vi "FuncVI_Sub - Probe - Master.vi"() -> ()   [LabVIEW 2021]
doc: "::: CalcExpress Toolkit :::\nCopyright (c) 2000-2026 Konstantin Shifershteyn. All rights reserved."
uses:
  cetypes.llb/CalcExpress Function Argument Info.ctl
  <vilib>/Utility/miscctls.llb/LVPointTypeDef.ctl
panel:
  out "I32B":i32 caption="Bit-keeping conversion" format="%.0x"
  in  "EnaWrap":bool=TRUE caption="Wrap Text"
  in  "ShowInt32":bool caption="show I32"
  out "I32M":i32 caption="Saturating conversion" format="%.0x"
  out "Index Range":cluster{"Initial index":i32, "Final index":i32}
  out "flattened data":string
  out "a2str":string[][](array[string])
  out "a1str":string[](array[string])
  out "a2cdb":cdb[][](array[numeric]) format="%.2f"
  out "a1cdb":cdb[](array[numeric]) format="%.2f"
  out "dbl":dbl format="%.2f"
  in  "update":bool
  in  "arg":T1
  out "a2dbl":dbl[][](array[numeric]) format="%.2f"
  out "cdb":cdb format="%.2f"
  out "a1dbl":dbl[](array[numeric]) format="%.2f"
  in  "Display style":u32(ring) items=["Normal", "'\\' Code", "Password", "Hex dump"]
  out "str":string
  in  "Precision":u8=3
  in  "Format":u8(ring) items=["Floating point", "Scientific", "Engineering", "Binary", "Octal", "Hexadecimal", "Relative time", "Absolute time"]
  out "datatype":u32(ring)=10 items=["String"=0, "DBL Number"=1, "Identifier"=2, "1D Array of DBL"=3, "2D Array of DBL"=4, "CDB Number"=5, "1D Array of CDB"=6, "2D Array of CDB"=7, "1D Array of String"=8, "2D Array of String"=9, "Unknown data type"=10, "Index Range"=252]
  # "Value:"
  # ":"
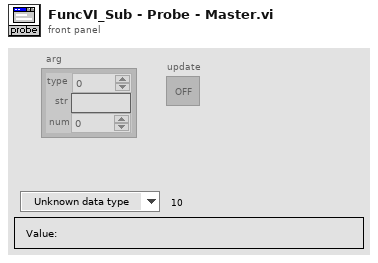
[diagram p1: front panel]
types:
  T1 = typedef "CalcExpress Function Argument Info.ctl" = cluster{"type":u32, "str":string, "num":dbl}
  T2 = typedef "LVPointTypeDef.ctl" = cluster{"Horizontal":i16, "Vertical":i16}
  T3 = typedef "eventvkey.ctl" = enum16{"ASCII", "Enter", "Return", "Shift", "Ctrl", "Alt", "Cmd", "Opt", "Caps", "NumLock", "Clear", "Break", "Up", "Down", "Left", "Right", "Insert", "Delete", "Home", "End", "PageUp", "PageDown", "Escape", "Help", "Pause", "ScrollLock", "F1", "F2", "F3", "F4", "F5", "F6", "F7", "F8", "F9", "F10", "F11", "F12", "F13", "F14", "F15", "F16", "F17", "F18", "F19", "F20", "F21", "F22", "F23", "F24", "Play", "VolumeUp", "VolumeDown", "Mute", "Two Byte Char"}
  T4 = cluster{"Shift":bool, "Ctrl":bool, "Alt":bool, "Cmd":bool, "Opt":bool}
  T5 = typedef "LVRectTypeDef.ctl" = cluster{"Left":i16, "Top":i16, "Right":i16, "Bottom":i16}
  T6 = cluster{"Left":i32, "Top":i32, "Right":i32, "Bottom":i32}
  T7 = typedef "LVPositionTypeDef.ctl" = cluster{"Left":i32, "Top":i32}
  T8 = typedef "LVBoundsTypeDef.ctl" = cluster{"Width":u32, "Height":u32}
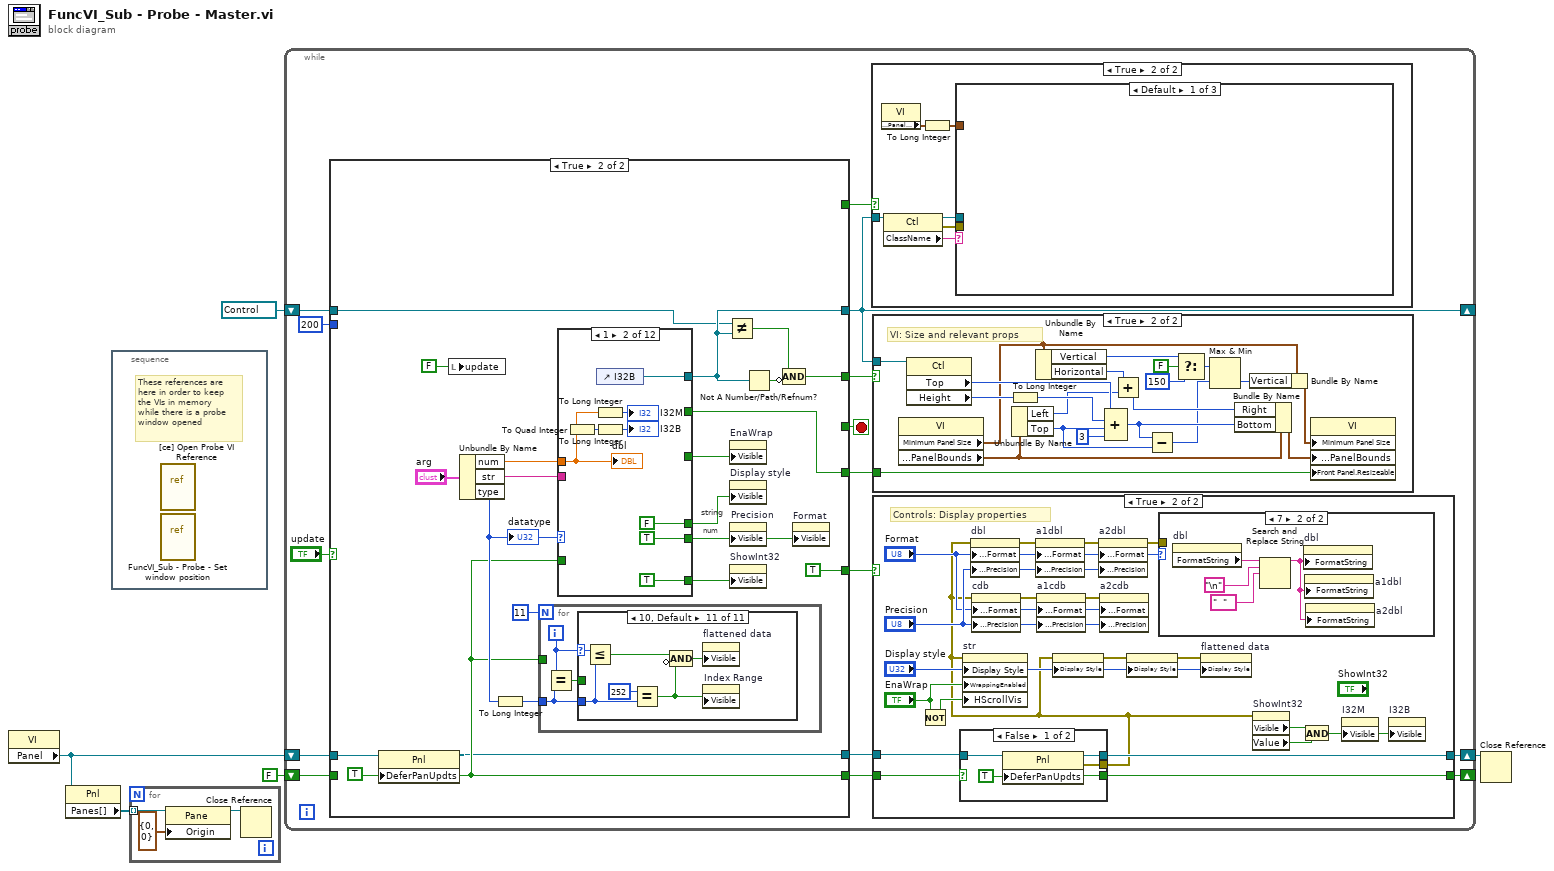
[diagram p0: block diagram]
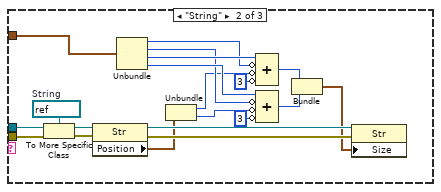
[diagram p3: hidden frame]
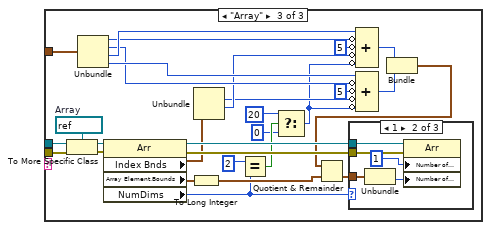
[diagram p4: hidden frame]
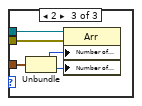
[diagram p6: hidden frame]
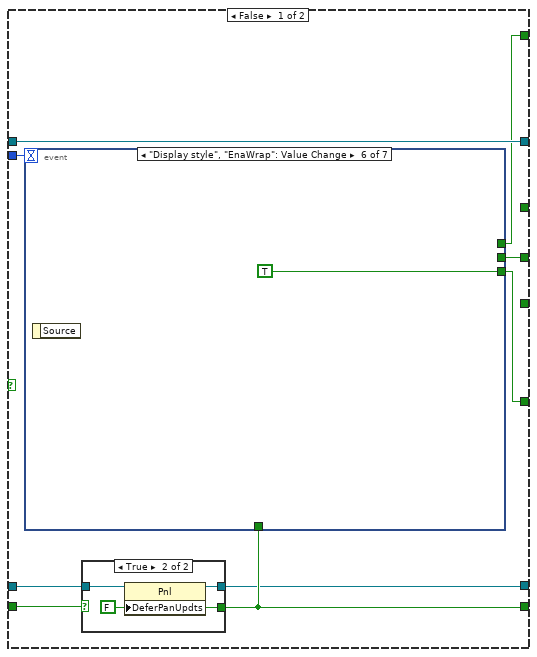
[diagram p8: hidden frame]
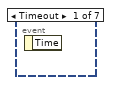
[diagram p10: hidden frame]
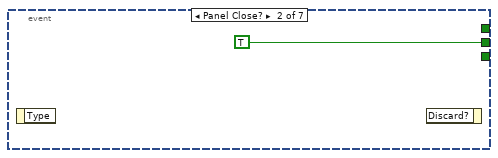
[diagram p11: hidden frame]
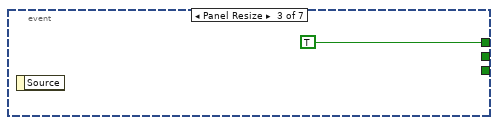
[diagram p12: hidden frame]
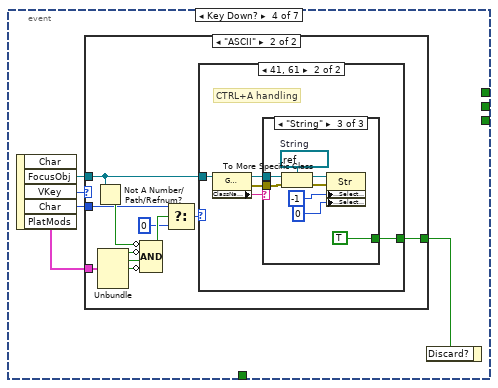
[diagram p13: hidden frame]
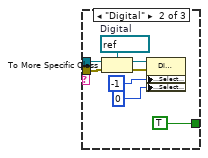
[diagram p17: hidden frame]
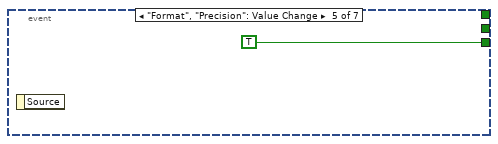
[diagram p18: hidden frame]
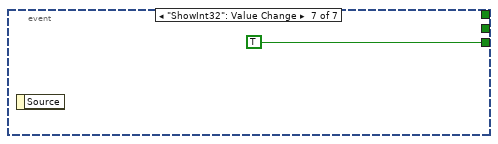
[diagram p19: hidden frame]
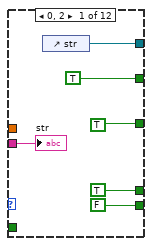
[diagram p20: hidden frame]
diagram:
  n1 = property on="Property Node" class="VI"() -> ("Panel"=w4:refnum<vi>)  [unwired: 2 in, 2 out]
  n2 = property on="Property Node" class="Pnl"(reference=w4) -> ("Panes[]"=w2:refnum<vi>[])  [unwired: 1 in, 2 out]
  n3 = stacked-sequence {
    frame #0 {
      # "These references are\nhere in order to keep\nthe VIs in memory\nwhile there is a probe\nwindow opened"
      n4 = vi-ref "[ce] Open Probe VI Reference.vi"() -> ()  [unwired: 1 out]
      n5 = vi-ref "FuncVI_Sub - Probe - Set window position.vi"() -> ()  [unwired: 1 out]
    }
  }
  n6 = for {
    tunnel: w2 -> [w8] mode=indexing
    n7 = property on="Property Node" class="Pane"(reference=w8, "Origin"=T2 {"Horizontal"=0, "Vertical"=0}) -> (reference out=w6:refnum<vi>)  [unwired: 1 in, 1 out]
    n8 = Close Reference(reference=w6) -> ()  [unwired: 1 in, 1 out]
  }
  n9 = while {
    shift-right: [w16] -> _
    shift-left: refnum<vi> refnum ("int32") -> [w18]
    shift-right: [w13] -> _
    shift-left: FALSE ("Defer Panel Updates") -> [w14]
    shift-right: [w10] -> w3
    shift-left: w4 -> [w15]
    stop <- w22 stop-if-true
    n10 = case shown="True" "update" {
      tunnel: [w118 _] -> w22
      tunnel: [w117 TRUE] -> w21
      tunnel: [w116 w173] -> w16
      tunnel: [_ w176] -> w20
      tunnel: [_ w174] -> w19
      tunnel: w18 -> [w116 w172]
      tunnel: [w115 _] -> w17
      tunnel: [w112 w169] -> w12
      tunnel: w15 -> [w114 w170]
      tunnel: w14 -> [w113 _]
      tunnel: [w111 w168] -> w11
      tunnel: 200 -> [w110 _]
      frame False {
        n11 = case shown="True" w113 {
          selector: w113 -> [w120 _]
          tunnel: w114 -> [w119 w123]
          tunnel: [w120 w122] -> w112
          tunnel: [w119 w121] -> w111
          frame False {
          }
          frame True {
            w122 = FALSE ("Defer Panel Updates")
            n12 = property on="Property Node" class="Pnl"(reference=w123, "DeferPanUpdts"=w122) -> (reference out=w121:refnum<vi>)  [unwired: 1 in, 1 out]
          }
        }
        n13 = event shown="[5] \"Display style\", \"EnaWrap\": Value Change" {
          selector: _ -> [_ _ _ _ _ _ _]
          dyn-events: _ -> [_ _ _ _ _ _ _]
          timeout: w110 -> [_ _ _ _ _ _ _]
          tunnel: [_ TRUE _ _ _ _ _] -> w118
          tunnel: [_ _ _ _ TRUE TRUE TRUE] -> w117
          tunnel: [_ _ TRUE _ _ _ _] -> w115
          tunnel: w112 -> [_ _ _ _ _ _ _]
          event Timeout {
            n14 = event-data() -> ()  [unwired: 1 in, 1 out]
          }
          event Panel Close? {
            n15 = event-data() -> ()  [unwired: 1 in, 1 out]
            n16 = event-data ("Event Filter Node")() -> ()  [unwired: 2 in, 1 out]
          }
          event Panel Resize {
            n17 = event-data() -> ()  [unwired: 1 in, 1 out]
          }
          event Key Down? {
            n18 = event-data() -> ("FocusObj"=w128:refnum<vi>, "VKey"=w130:T3, "Char"=w127:i16, "PlatMods"=w129:T4)  [unwired: 1 in, 1 out]
            n19 = case shown="\"ASCII\"" w130 {
              tunnel: w129 -> [_ w137]
              tunnel: w128 -> [_ w136]
              tunnel: w127 -> [_ w135]
              tunnel: [_ w131] -> w126
              frame Default {
              }
              frame "ASCII" {
                n20 = Not A Number/Path/Refnum?(number/path/refnum=w136) -> (NaN/Path/Refnum?=w138:bool)
                n21 = Unbundle(w137) -> ("Shift"=w139:bool, "Ctrl"=w140:bool, "Alt"=w141:bool)  [unwired: 2 out]
                n22 = Compound Arithmetic op=AND(invert w138, invert w139, w140, invert w141) -> (w134:bool)
                n23 = Select(t=w135, s=w134, f=i16 0) -> (s? t:f=w132:i16)
                n24 = case shown="41, 61" w132 {
                  tunnel: w136 -> [_ w146]
                  tunnel: [_ w142] -> w131
                  frame Default {
                  }
                  frame 65, 97 {
                    # "CTRL+A handling"
                    n25 = property on="Property Node" class="GObj"(reference=w146) -> (reference out=w144:refnum<vi>, error out=w143:errorcluster, "ClassName"=w145:string)  [unwired: 1 in]
                    n26 = case shown="\"String\"" w145 {
                      tunnel: w144 -> [_ w150 w158]
                      tunnel: w143 -> [_ w149 w157]
                      tunnel: [_ TRUE TRUE] -> w142
                      frame Default {
                      }
                      frame "Digital" {
                        w151 = refnum<vi> refnum  # Digital
                        n27 = To More Specific Class(target class=w151, reference=w150, error in=w149) -> (specific class reference=w154:refnum<vi>, error out=w148:errorcluster)
                        n28 = property on="Property Node" class="DigNum"(reference=w154, error in=w148, "NumText.Selection End"=-1 ("Numeric Text.Selection:End"), "NumText.Selection Start"=u32 0 ("Numeric Text.Selection:Start")) -> ()  [unwired: 2 out]
                      }
                      frame "String" {
                        w159 = refnum<vi> refnum  # String
                        n29 = To More Specific Class(target class=w159, reference=w158, error in=w157) -> (specific class reference=w162:refnum<vi>, error out=w156:errorcluster)
                        n30 = property on="Property Node" class="Str"(reference=w162, error in=w156, "Text.Selection End"=-1 ("Numeric Text.Selection:End"), "Text.Selection Start"=u32 0 ("Numeric Text.Selection:Start")) -> ()  [unwired: 2 out]
                      }
                    }
                  }
                }
              }
            }
            n31 = event-data ("Event Filter Node")("Discard?"=w126) -> ()  [unwired: 1 in, 1 out]
          }
          event "Format", "Precision": Value Change {
            n32 = event-data() -> ()  [unwired: 1 in, 1 out]
          }
          event "Display style", "EnaWrap": Value Change {
            n33 = event-data() -> ()  [unwired: 1 in, 1 out]
          }
          event "ShowInt32": Value Change {
            n34 = event-data() -> ()  [unwired: 1 in, 1 out]
          }
        }
      }
      frame True {
        w169 = TRUE
        # "num"
        # "string"
        n35 = property on="Property Node" class="Pnl"(reference=w170, "DeferPanUpdts"=w169) -> (reference out=w168:refnum<vi>)  [unwired: 1 in, 1 out]
        n36 = local write "update"(FALSE ("update")) -> ()
        n37 = Unbundle By Name("arg") -> ("num"=w184:dbl, "str"=w185:string, "type"=w179:u32)
        "datatype" <- w179
        n38 = To Long Integer(number=w179) -> (32bit integer=w183:i32)
        n39 = for {
          N: 11 -> [_]
          tunnel: w183 -> [w262]
          tunnel: w169 -> [_]
          i -> [w263]
          n40 = Equal?(x=w263, y=w262) -> (x = y?=w264:bool)
          n41 = case shown="10, Default" w263 {
            selector: w263 -> [_ _ _ _ _ _ _ _ _ _ w279]
            tunnel: w264 -> [w265 w266 _ w267 w268 w269 w270 w271 w272 w273 _]
            tunnel: w262 -> [_ _ _ _ _ _ _ _ _ _ w278]
            frame 0 {
              n42 = property on="str" class="Str"("Visible"=w265) -> ()  [unwired: 2 in, 2 out]
            }
            frame 1 {
              n43 = property on="dbl" class="DigNum (strict)"("Visible"=w266) -> ()  [unwired: 2 in, 2 out]
            }
            frame 2 {
            }
            frame 3 {
              n44 = property on="a1dbl" class="Arr (strict)"("Visible"=w267) -> ()  [unwired: 2 in, 2 out]
            }
            frame 4 {
              n45 = property on="a2dbl" class="Arr (strict)"("Visible"=w268) -> ()  [unwired: 2 in, 2 out]
            }
            frame 5 {
              n46 = property on="cdb" class="DigNum (strict)"("Visible"=w269) -> ()  [unwired: 2 in, 2 out]
            }
            frame 6 {
              n47 = property on="a1cdb" class="Arr (strict)"("Visible"=w270) -> ()  [unwired: 2 in, 2 out]
            }
            frame 7 {
              n48 = property on="a2cdb" class="Arr (strict)"("Visible"=w271) -> ()  [unwired: 2 in, 2 out]
            }
            frame 8 {
              n49 = property on="a1str" class="Arr (strict)"("Visible"=w272) -> ()  [unwired: 2 in, 2 out]
            }
            frame 9 {
              n50 = property on="a2str" class="Arr (strict)"("Visible"=w273) -> ()  [unwired: 2 in, 2 out]
            }
            frame 10, Default {
              n51 = Less Or Equal?(x=w279, y=w278) -> (x <= y?=w274:bool)
              n52 = Equal?(x=252, y=w278) -> (x = y?=w275:bool)
              n53 = Compound Arithmetic op=AND(w274, invert w275) -> (w276:bool)
              n54 = property on="flattened data" class="Str"("Visible"=w276) -> ()  [unwired: 2 in, 2 out]
              n55 = property on="Index Range" class="Clust (strict)"("Visible"=w275) -> ()  [unwired: 2 in, 2 out]
            }
          }
        }
        n56 = case shown="1" w179 {
          tunnel: w184 -> [_ w193 _ _ _ _ _ _ _ _ _ w261]
          tunnel: [FALSE TRUE FALSE TRUE TRUE TRUE TRUE TRUE FALSE FALSE FALSE FALSE] -> w181
          tunnel: [TRUE FALSE FALSE FALSE FALSE FALSE FALSE FALSE TRUE TRUE TRUE FALSE] -> w167
          tunnel: w185 -> [w190 _ _ w208 w215 w221 w228 w234 w242 w248 w254 _]
          tunnel: [_ TRUE _ _ _ _ _ _ _ _ _ _] -> w177
          tunnel: [w189 w196 refnum<vi> refnum ("int32") w205 w212 w218 w225 w232 w239 w246 w253 w257] -> w173
          tunnel: [TRUE _ _ TRUE TRUE _ TRUE TRUE TRUE TRUE TRUE _] -> w174
          tunnel: w169 -> [_ _ _ _ _ _ _ _ _ _ _ _]
          tunnel: [TRUE _ _ _ _ _ _ _ _ _ _ _] -> w166
          frame 0, 2 {
            n57 = control-ref of="str"() -> (w189:refnum<vi>)
            "str" <- w190
          }
          frame 1 {
            n58 = To Quad Integer(1:w193) -> (0:w194:i64)
            n59 = To Long Integer(number=w193) -> (32bit integer=→"I32M":i32)
            n60 = To Long Integer(number=w194) -> (32bit integer=→"I32B":i32)
            n61 = control-ref of="I32B"() -> (w196:refnum<vi>)
            "dbl" <- w193
          }
          frame 22222 {
          }
          frame 3 {
            n62 = control-ref of="a1dbl"() -> (w205:refnum<vi>)
            n63 = Unflatten From String(type=dbl[] [] ("a1dbl"), binary string=w208) -> (value=→"a1dbl":dbl[])  [unwired: 3 in, 2 out]
          }
          frame 4 {
            n64 = control-ref of="a2dbl"() -> (w212:refnum<vi>)
            n65 = Unflatten From String(type=dbl[][] [] ("a1dbl"), binary string=w215) -> (value=→"a2dbl":dbl[][])  [unwired: 3 in, 2 out]
          }
          frame 5 {
            n66 = control-ref of="cdb"() -> (w218:refnum<vi>)
            n67 = Unflatten From String(type=cdb 0.0+0.0i ("cdb"), binary string=w221) -> (value=→"cdb":cdb)  [unwired: 3 in, 2 out]
          }
          frame 6 {
            n68 = control-ref of="a1cdb"() -> (w225:refnum<vi>)
            n69 = Unflatten From String(type=cdb[] [] ("a1dbl"), binary string=w228) -> (value=→"a1cdb":cdb[])  [unwired: 3 in, 2 out]
          }
          frame 7 {
            n70 = Unflatten From String(type=cdb[][] [] ("a1dbl"), binary string=w234) -> (value=→"a2cdb":cdb[][])  [unwired: 3 in, 2 out]
            n71 = control-ref of="a2cdb"() -> (w232:refnum<vi>)
          }
          frame 8 {
            n72 = control-ref of="a1str"() -> (w239:refnum<vi>)
            n73 = Unflatten From String(type=string[] [] ("a1str"), binary string=w242) -> (value=→"a1str":string[])  [unwired: 3 in, 2 out]
          }
          frame 9 {
            n74 = control-ref of="a2str"() -> (w246:refnum<vi>)
            n75 = Unflatten From String(type=string[][] [] ("a1str"), binary string=w248) -> (value=→"a2str":string[][])  [unwired: 3 in, 2 out]
          }
          frame 10, Default {
            n76 = control-ref of="flattened data"() -> (w253:refnum<vi>)
            "flattened data" <- w254
          }
          frame 252 {
            n77 = call "[ce] Index Range to-from DBL.vi"("dbl scalar"=w261) -> ("Index Range out"=→"Index Range":cluster{"Initial index":i32, "Final index":i32})  [unwired: 9 in, 1 out]
            n78 = control-ref of="Index Range"() -> (w257:refnum<vi>)
          }
        }
        n79 = Not Equal?(x=w172, y=w173) -> (x != y?=w171:bool)
        n80 = property on="EnaWrap" class="Bool (strict)"("Visible"=w166) -> ()  [unwired: 2 in, 2 out]
        n81 = property on="Display style" class="Ring (strict)"("Visible"=w167) -> ()  [unwired: 2 in, 2 out]
        n82 = property on="Precision" class="DigNum (strict)"("Visible"=w181) -> ()  [unwired: 2 in, 2 out]
        n83 = property on="ShowInt32" class="Bool (strict)"("Visible"=w177) -> ()  [unwired: 2 in, 2 out]
        n84 = Not A Number/Path/Refnum?(number/path/refnum=w173) -> (NaN/Path/Refnum?=w175:bool)
        n85 = Compound Arithmetic op=AND(w171, invert w175) -> (w176:bool)
        n86 = property on="Format" class="Ring (strict)"("Visible"=w181) -> ()  [unwired: 2 in, 2 out]
      }
    }
    n87 = case shown="True" w17 {
      tunnel: w16 -> [_ w29]
      frame False {
      }
      frame True {
        n88 = property on="Property Node" class="VI"() -> ("Front Panel.PanelBounds"=w25:T5)  [unwired: 2 in, 2 out]
        n89 = property on="Property Node" class="Ctl"(reference=w29) -> (reference out=w27:refnum<vi>, error out=w26:errorcluster, "ClassName"=w28:string)  [unwired: 1 in]
        n90 = To Long Integer(number=w25) -> (32bit integer=w24:T6)
        n91 = case shown="Default" w28 {
          tunnel: w27 -> [_ w49 w78]
          tunnel: w26 -> [_ w34 w69]
          tunnel: w24 -> [_ w31 w66]
          frame Default {
          }
          frame "String" {
            w48 = refnum<vi> refnum  # String
            n92 = To More Specific Class(target class=w48, reference=w49, error in=w34) -> (specific class reference=w33:refnum<vi>, error out=w32:errorcluster)
            n93 = property on="Property Node" class="Str"(reference=w33, error in=w32) -> (reference out=w46:refnum<vi>, error out=w47:errorcluster, "Position"=w45:T7)
            n94 = Unbundle(w31) -> ("Left"=w30:i32, "Top"=w42:i32, "Right"=w44:i32, "Bottom"=w43:i32)
            n95 = Unbundle(w45) -> ("Left"=w41:i32, "Top"=w40:i32)
            n96 = Compound Arithmetic op=ADD(w44, invert w30, invert w41, invert 3 ("value")) -> (w39:i32)
            n97 = Compound Arithmetic op=ADD(w43, invert w42, invert w40, invert 3 ("value")) -> (w38:i32)
            n98 = Bundle(w39, w38) -> (w37:cluster{i32, i32})  [unwired: 1 in]
            n99 = property on="Property Node" class="Str"(reference=w46, error in=w47, "Size"=w37) -> ()  [unwired: 2 out]
          }
          frame "Array" {
            w77 = refnum<vi> refnum  # Array
            n100 = To More Specific Class(target class=w77, reference=w78, error in=w69) -> (specific class reference=w68:refnum<vi>, error out=w67:errorcluster)
            n101 = Unbundle(w66) -> ("Left"=w65:i32, "Top"=w72:i32, "Right"=w74:i32, "Bottom"=w73:i32)
            n102 = property on="Property Node" class="Arr"(reference=w68, error in=w67) -> (reference out=w75:refnum<vi>, error out=w76:errorcluster, "Index Bnds"=w59:T5, "Array Element.Bounds"=w64:T8, "NumDims"=w51:u32)
            n103 = To Long Integer(number=w64) -> (32bit integer=w61:cluster{"Width":i32, "Height":i32})
            n104 = Unbundle(w59) -> ("Top"=w57:i16, "Right"=w58:i16)  [unwired: 2 out]
            n105 = Equal?(x=u32 2 ("y"), y=w51) -> (x = y?=w55:bool)
            n106 = Select(t=20 ("value"), s=w55, f=0) -> (s? t:f=w50:i32)
            n107 = Compound Arithmetic op=ADD(w74, invert w65, invert 5 ("value"), invert w58, invert w50) -> (w71:i32)
            n108 = Compound Arithmetic op=ADD(w73, invert w72, invert 5 ("value"), invert w57, invert w50) -> (w70:i32)
            n109 = Bundle(w71, w70) -> (w56:cluster{i32, i32})  [unwired: 1 in]
            n110 = Quotient & Remainder(x=w56, y=w61) -> (floor(x/y)=w60:cluster{i32, i32})  [unwired: 1 out]
            n111 = case shown="1" w51 {
              tunnel: w76 -> [_ w83 w88]
              tunnel: w75 -> [_ w82 w87]
              tunnel: w60 -> [_ w81 w86]
              frame 0, Default {
              }
              frame 1 {
                n112 = Unbundle(w81) -> (w80:i32)  [unwired: 1 out]
                n113 = property on="Property Node" class="Arr"(reference=w82, error in=w83, "Number of Columns"=u32 1, "Number of Rows"=w80) -> ()  [unwired: 2 out]
              }
              frame 2 {
                n114 = Unbundle(w86) -> (w85:i32, w84:i32)
                n115 = property on="Property Node" class="Arr"(reference=w87, error in=w88, "Number of Columns"=w85, "Number of Rows"=w84) -> ()  [unwired: 2 out]
              }
            }
          }
        }
      }
    }
    n116 = case shown="True" w20 {
      tunnel: w16 -> [_ w109]
      tunnel: w19 -> [_ w97]
      frame False {
      }
      frame True {
        # "VI: Size and relevant props"
        n117 = property on="Property Node" class="VI"() -> ("Minimum Panel Size"=w96:T2, "Front Panel.PanelBounds"=w104:T5)  [unwired: 2 in, 2 out]
        n118 = property on="Property Node" class="Ctl"(reference=w109) -> ("Top"=w108:i32, "Height"=w107:u32)  [unwired: 1 in, 2 out]
        n119 = To Long Integer(number=w107) -> (32bit integer=w106:i32)
        n120 = Unbundle By Name(w104) -> ("Left"=w101:i16, "Top"=w98:i16)
        n121 = Unbundle By Name(w96) -> ("Vertical"=w92:i16, "Horizontal"=w102:i16)
        n122 = Compound Arithmetic op=ADD(w108, w106, w98, 3 ("value")) -> (w99:i32)
        n123 = Add(x=w102, y=w101) -> (x+y=w100:i16)
        n124 = Subtract(x=w99, y=w98) -> (x-y=w93:i32)
        n125 = Select(t=w92, s=FALSE, f=150 ("x")) -> (s? t:f=w90:i32)
        n126 = Max & Min(x=w90, y=w93) -> (min(x,y)=w94:i32)  [unwired: 1 out]
        n127 = Bundle By Name(cluster=w104, "Right"=w100, "Bottom"=w99) -> (w103:T5)
        n128 = Bundle By Name(cluster=w96, "Vertical"=w94) -> (w95:T2)
        n129 = property on="Property Node" class="VI"("Minimum Panel Size"=w95, "Front Panel.PanelBounds"=w103, "Front Panel.Resizeable"=w97) -> ()  [unwired: 2 in, 2 out]
      }
    }
    n130 = case shown="True" w21 {
      tunnel: [w281 w293] -> w13
      tunnel: w12 -> [w281 w294]
      tunnel: w11 -> [w280 w295]
      tunnel: [w280 w284] -> w10
      frame False {
      }
      frame True {
        # "Controls: Display properties"
        n131 = Not(x="EnaWrap") -> (.not. x?=w285:bool)
        n132 = case shown="False" w294 {
          selector: w294 -> [_ w307]
          tunnel: w295 -> [w305 w306]
          tunnel: [w304 w307] -> w293
          tunnel: [w303 w306] -> w284
          tunnel: [w302 _] -> w283
          frame False {
            w304 = TRUE ("Defer Panel Updates")
            n133 = property on="Property Node" class="Pnl"(reference=w305, "DeferPanUpdts"=w304) -> (reference out=w303:refnum<vi>, error out=w302:errorcluster)  [unwired: 1 in]
          }
          frame True {
          }
        }
        n134 = property on="str" class="Str"(error in=w283, "Display Style"="Display style", "WrappingEnabled"="EnaWrap", "HScrollVis"=w285) -> ()  [unwired: 1 in, 2 out]
        n135 = property on="dbl" class="DigNum (strict)"(error in=w283, "Display Format:Format"="Format", "Display Format:Precision"="Precision") -> (error out=w292:errorcluster)  [unwired: 1 in, 1 out]
        n136 = property on="cdb" class="DigNum (strict)"(error in=w283, "Display Format:Format"="Format", "Display Format:Precision"="Precision") -> (error out=w290:errorcluster)  [unwired: 1 in, 1 out]
        n137 = property on="a1dbl" class="DigNum (strict)"(error in=w292, "Display Format:Format"="Format", "Display Format:Precision"="Precision") -> (error out=w291:errorcluster)  [unwired: 1 in, 1 out]
        n138 = property on="a1cdb" class="DigNum (strict)"(error in=w290, "Display Format:Format"="Format", "Display Format:Precision"="Precision") -> (error out=w289:errorcluster)  [unwired: 1 in, 1 out]
        n139 = property class="Str"(error in=w283, "Display Style"="Display style") -> (error out=w288:errorcluster)  [unwired: 1 in, 1 out]
        n140 = property on="a2dbl" class="DigNum (strict)"(error in=w291, "Display Format:Format"="Format", "Display Format:Precision"="Precision") -> (error out=w296:errorcluster)  [unwired: 1 in, 1 out]
        n141 = property on="a2cdb" class="DigNum (strict)"(error in=w289, "Display Format:Format"="Format", "Display Format:Precision"="Precision") -> ()  [unwired: 1 in, 2 out]
        n142 = property class="Str"(error in=w288, "Display Style"="Display style") -> (error out=w287:errorcluster)  [unwired: 1 in, 1 out]
        n143 = case shown="7" "Format" {
          tunnel: w296 -> [_ _]
          frame 0, Default {
          }
          frame 7 {
            n144 = property on="dbl" class="DigNum (strict)"() -> ("FormatString"=w311:string)  [unwired: 2 in, 2 out]
            n145 = Search and Replace String(input string=w311, search string="\n" ("Line Feed Constant"), replace string="  ") -> (result string=w310:string)  [unwired: 5 in, 3 out]
            n146 = property on="dbl" class="DigNum (strict)"("FormatString"=w310) -> ()  [unwired: 2 in, 2 out]
            n147 = property on="a1dbl" class="DigNum (strict)"("FormatString"=w310) -> ()  [unwired: 2 in, 2 out]
            n148 = property on="a2dbl" class="DigNum (strict)"("FormatString"=w310) -> ()  [unwired: 2 in, 2 out]
          }
        }
        n149 = property on="flattened data" class="Str"(error in=w287, "Display Style"="Display style") -> ()  [unwired: 1 in, 2 out]
        n150 = property on="ShowInt32" class="Bool (strict)"(error in=w283) -> ("Visible"=w299:bool, "Value"=w298:bool)  [unwired: 1 in, 2 out]
        n151 = And(x=w299, y=w298) -> (x .and. y?=w282:bool)
        n152 = property on="I32M" class="DigNum (strict)"("Visible"=w282) -> ()  [unwired: 2 in, 2 out]
        n153 = property on="I32B" class="DigNum (strict)"("Visible"=w282) -> ()  [unwired: 2 in, 2 out]
      }
    }
  }
  n154 = Close Reference(reference=w3) -> ()  [unwired: 1 in, 1 out]
